vi "Read Device ID.vi"(8 "error in (no error)":errorcluster, 11 "Device":string="hidraw0") -> (0 "error out":errorcluster, 3 "Relay ID":T1 {"Serial Number" format="%06x"})   [LabVIEW 2021, in "USB Relay Control.lvlib"]
uses:
  USB Relay Control.lvlib
  typedef/Relay ID.ctl
  typedef/Read Write.ctl
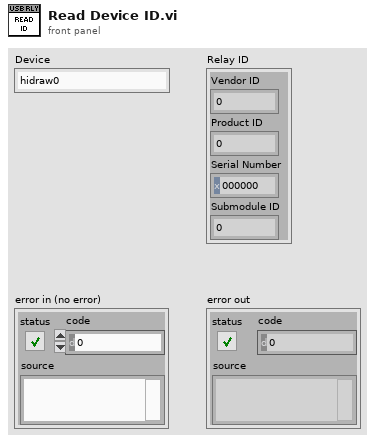
[diagram p1: front panel]
types:
  T1 = typedef "USB Relay Control.lvlib/Relay ID.ctl" = cluster{"Vendor ID":u8, "Product ID":u8, "Serial Number":u32, "Submodule ID":u8}
  T2 = typedef "USB Relay Control.lvlib/Read Write.ctl" = enum8{"Read", "Write"}
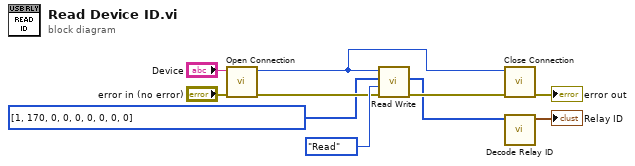
[diagram p0: block diagram]
diagram:
  n1 = call "Open Connection.vi"("error in (no error)"="error in (no error)", "Device"="Device") -> ("error out"=w2:errorcluster, "HID Handle"=w9:i64)  [unwired: 8 in]
  n2 = call "Read Write.vi"("error in (no error)"=w2, "RW"=Read_Write."Read", "Buffer In"=u8[] [1, 170, 0, 0, 0, 0, 0, 0, 0], "HID Handle"=w9) -> ("error out"=w10:errorcluster, "Buffer Out"=w3:u8[])  [unwired: 6 in]
  n3 = call "Close Connection.vi"("error in (no error)"=w10, "HID Handle"=w9) -> ("error out"=→"error out":errorcluster)  [unwired: 9 in]
  n4 = call "Decode Relay ID.vi"("Encoded ID"=w3) -> ("Relay ID"=→"Relay ID":T1)  [unwired: 10 in]
